vi "CSM - Generate User Global Log.vi"(5 "Userlog Name (\"\" as default)":string, 6 "From Who":string, 7 "Place (\"\" to Use VI's Name)":string, 8 "Error In":errorcluster caption="error in (no error)", 10 "Arguments":string, 11 "Log":string) -> (0 "error out":errorcluster)   [LabVIEW 2017, in "Communicable State Machine.lvlib"]
doc: "Generates a custom user log for scenarios such as debugging. When the input parameters of this VI contain error information, CSM - Global Log Error Handler VI is called to record the error information.\n\n> [!NOTE] <b>Custom User Name</b>\n>\n> Users can customize the name of the user log. The default is [User Log].\n>\n> For example: when the user does not customize the name, the default [User Log] is used. When the user customizes the name to [MYLOG], the log will be displayed as [MYLOG]. The comparison is as follows:\n>\n> 14:55:59.676 [14:55:59.676] [User Log] Module | Value >> 0.487854\n> 14:55:59.676 [14:55:59.676] [MYLOG] Module | Value >> 0.487854\n\n-- <b>Controls</b> --\n- <b>Log</b>: Event name.\n- <b>Arguments</b>: Event arguments.\n- <b>From Who</b>: Source.\n- <b>ModuleName</b>: Module name.\n- <b>Place (\"\" to Use VI's Name)</b>: Location where the error occurred. The default is the name of the VI.\n- <b>UserLog Name(\"\" as Default)</b>: User log name. The default is \"User Log\"."
uses:
  Communicable State Machine.lvlib
  _Support/Typedef/_CSM_GlobalLog_MSG.ctl
  _Support/Typedef/_CSM_Response Source Message.ctl
  _Support/Typedef/_CSM_GlobalLog_MSG_TYPE.ctl
  CSM - Make String Arguments Safe.vi
  _Support/GlobalEvent/GEvt-Convert Filter Rules - v1.2.vi
  _Support/ChangeFlag/FlagInstance-GEvt Filter.vi
  _Support/ChangeFlag/FlagInstance-GEvt Refs.vi
  CSM - Keywords.vi
  _Support/ChangeFlag/ChangeFlag-Read.vi
  _Support/GlobalEvent/LogFilter/LogFilter - Check.vi
  _Support/GlobalEvent/LogFilter/SettingVIs/Set Periodic Log Filter.vi
  _Support/GlobalEvent/LogFilter/SettingVIs/Set CSM UserLog Filter.vi
  _Support/GlobalEvent/LogFilter/SettingVIs/Set CSM Broadcast Filter.vi
  _Support/GlobalEvent/LogFilter/SettingVIs/Set CSM StateType Filter.vi
  _Support/GlobalEvent/LogFilter/SettingVIs/Set Global StateType Filter.vi
  _Support/GlobalEvent/LogFilter/SettingVIs/Set CSM State Filter.vi
  _Support/GlobalEvent/LogFilter/SettingVIs/Set CSM LogType Filter.vi
  _Support/GlobalEvent/LogFilter/SettingVIs/Set Global UserLog Filter.vi
  _Support/GlobalEvent/LogFilter/SettingVIs/Set Global Broadcast Filter.vi
  _Support/GlobalEvent/LogFilter/SettingVIs/Set Global State Filter.vi
  _Support/GlobalEvent/LogFilter/SettingVIs/Set Global LogType Filter.vi
  _Support/GlobalEvent/LogFilter/SettingVIs/Set Global CSM Filter.vi
  _Support/GlobalEvent/FGV-GEvt Filter Rules(lvlibp).vi
  _Support/ChangeFlag/ChangeFlagDB.vi
  _Support/GlobalEvent/GEvt-Valid Subscribers.vi
  _Support/GlobalEvent/FGV-GlobalEventQueues(lvlibp).vi
  _Support/GlobalEvent/FGV-GlobalEventRef(lvlibp).vi
  _Support/GlobalEvent/LogFilter/LogFilter.lvclass
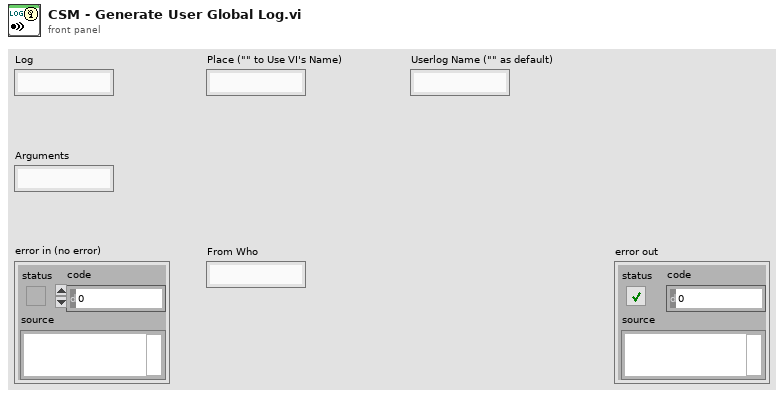
[diagram p1: front panel]
types:
  T1 = typedef "Communicable State Machine.lvlib/GEvt-Refs.ctl" = cluster{"Event":refnum<user-event>, "Queues":refnum<queue>[], "Valid":bool}
  T2 = typedef "Communicable State Machine.lvlib/_CSM_GlobalLog_MSG_TYPE.ctl" = enum16{"User Log", "State Change", "Status", "Interrupt", "Register", "Unregister", "Error Log", "Module Created", "Module Destroyed", "Async Message", "No-Rep Async Message", "Sync Message", "AsyncMsg Complete", "SyncMsg Complete"}
  T3 = typedef "Communicable State Machine.lvlib/_CSM_GlobalLog_MSG.ctl" = cluster{"Name (\"\" to Use UUID)":string, "Current State":string, "Arguments":string, "Source Message":T4, "Source Module":string, "Complete(T)/Start(F)":bool, "LogType":T2, "Time Stamp":timestamp}
  T4 = typedef "Communicable State Machine.lvlib/_CSM_Response Source Message.ctl" = cluster{"‘State":string, "’Arguments":string, "’Error":errorcluster}
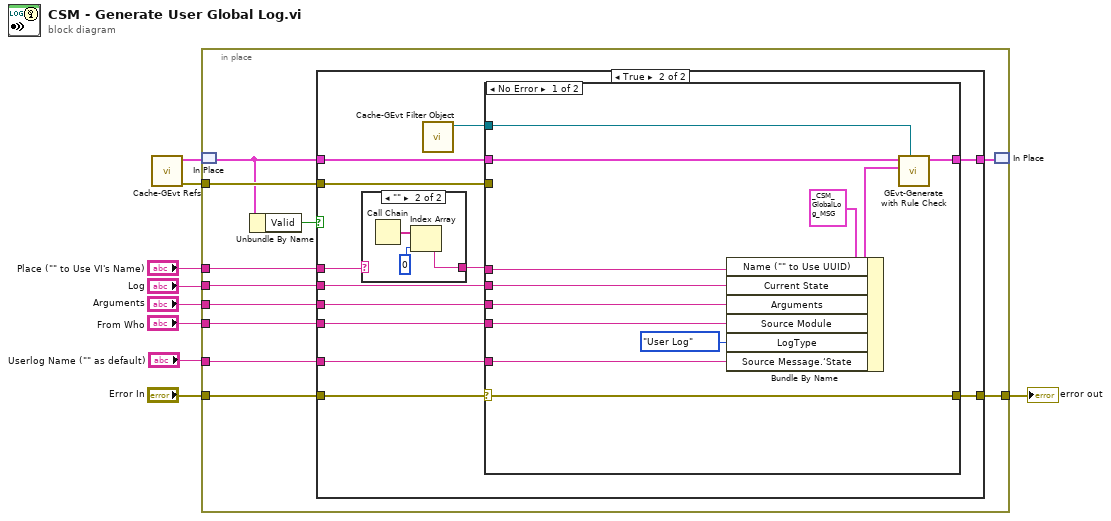
[diagram p0: block diagram]
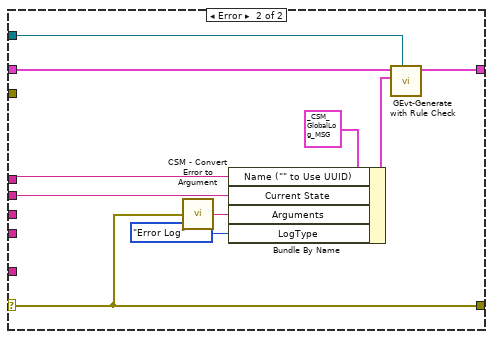
[diagram p4: hidden frame]
diagram:
  n1 = call "Cache-GEvt Refs.vi"() -> ("error out"=w2:errorcluster, "CSM Global Log Ref"=w3:T1)  [unwired: 10 in]
  n2 = in-place {
    in-place-border: "Place (\"\" to Use VI's Name)" -> [w19]
    in-place-border: "Log" -> [w18]
    in-place-border: "Arguments" -> [w17]
    in-place-border: w2 -> [w16]
    in-place-border: [w15] -> w9
    in-place-border: "From Who" -> [w14]
    in-place-border: "Error In" -> [w13]
    in-place-border: "Userlog Name (\"\" as default)" -> [w10]
    n3 = in-place-match #1(w3) -> (w12:T1)
    n4 = Unbundle By Name(w12) -> ("Valid"=w11:bool)
    n5 = case shown="True" w11 {
      tunnel: w12 -> [w22 w34]
      tunnel: w19 -> [_ w26]
      tunnel: [w22 w33] -> w20
      tunnel: w18 -> [_ w32]
      tunnel: w17 -> [_ w31]
      tunnel: w16 -> [w21 w30]
      tunnel: [w21 w29] -> w15
      tunnel: w14 -> [_ w28]
      tunnel: w13 -> [_ w27]
      tunnel: w10 -> [_ w23]
      frame False {
      }
      frame True {
        n6 = case shown="\"\"" w26 {
          selector: w26 -> [w35 _]
          tunnel: [w35 w36] -> w25
          frame Default {
          }
          frame "" {
            n7 = Call Chain() -> (call chain=w37:string[])
            n8 = Index Array(array=w37, index=0 ("Index")) -> (element=w36:string)
          }
        }
        n9 = call "Cache-GEvt Filter Object.vi"() -> ("CSM:LogFilter.lvclass"=w24:refnum<class "LogFilter.lvclass">)  [unwired: 11 in]
        n10 = case shown="No Error" w27 {
          selector: w27 -> [w42 w58]
          tunnel: w34 -> [w50 w60]
          tunnel: [w47 w59] -> w33
          tunnel: w32 -> [w46 w53]
          tunnel: w31 -> [w45 _]
          tunnel: w30 -> [_ _]
          tunnel: [w42 w58] -> w29
          tunnel: w28 -> [w43 _]
          tunnel: w25 -> [w41 w52]
          tunnel: w24 -> [w40 w51]
          tunnel: w23 -> [w39 _]
          frame No Error {
            n11 = Bundle By Name(cluster=T3 {"Name (\"\" to Use UUID)"="", "Current State"="", "Arguments"="", "Source Message"={"‘State"="", "’Arguments"="", "’Error"={"status"=FALSE, "code"=0, "source"=""}}, "Source Module"="", "Complete(T)/Start(F)"=FALSE, "LogType"=enum."User Log", "Time Stamp"=timestamp(0 s since 1904-01-01)} ("event data"), "Name (\"\" to Use UUID)"=w41, "Current State"=w46, "Arguments"=w45, "Source Module"=w43, "LogType"=_CSM_GlobalLog_MSG_TYPE."User Log" ("Type"), "Source Message.‘State"=w39) -> (w48:T3)
            n12 = call "GEvt-Generate with Rule Check.vi"("LogFilter In"=w40, "Event Data"=w48, "CSM Global Log Event In"=w50) -> ("CSM Global Log Event Out"=w47:T1)  [unwired: 8 in]
          }
          frame Error {
            n13 = call "CSM - Convert Error to Argument.vi"("Error"=w58) -> ("Argument"=w54:string)  [unwired: 4 in]
            n14 = Bundle By Name(cluster=T3 {"Name (\"\" to Use UUID)"="", "Current State"="", "Arguments"="", "Source Message"={"‘State"="", "’Arguments"="", "’Error"={"status"=FALSE, "code"=0, "source"=""}}, "Source Module"="", "Complete(T)/Start(F)"=FALSE, "LogType"=enum."User Log", "Time Stamp"=timestamp(0 s since 1904-01-01)} ("event data"), "Name (\"\" to Use UUID)"=w52, "Current State"=w53, "Arguments"=w54, "LogType"=_CSM_GlobalLog_MSG_TYPE."Error Log" ("Type")) -> (w56:T3)
            n15 = call "GEvt-Generate with Rule Check.vi"("LogFilter In"=w51, "Event Data"=w56, "CSM Global Log Event In"=w60) -> ("CSM Global Log Event Out"=w59:T1)  [unwired: 8 in]
          }
        }
      }
    }
    n16 = in-place-match #1(w20) -> ()  [unwired: 1 out]
  }
  "error out" <- w9
